vi "Test JKI SM Helper.vi"() -> ()   [LabVIEW 2020]
uses:
  source/JKI State Machine API/source/JKI SM/JKI SM.lvclass/JKI SM.ctl
  source/JKI State Machine API/source/JKI SM/JKI SM.lvclass
  source/JKI State Machine API/tests/TEST JKI State Machine API.lvlib
panel:
  out "error out":errorcluster
  in  "EventStructure?":bool
  # "Run this VI to lauch the JKI State Machine helper on a template VI"
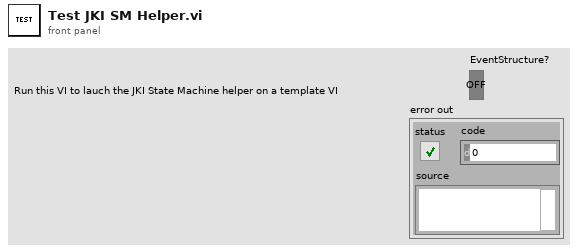
[diagram p1: front panel]
types:
  T1 = cluster{"App.ContextName":string, "VI.Name":string, "Object UID":i32}
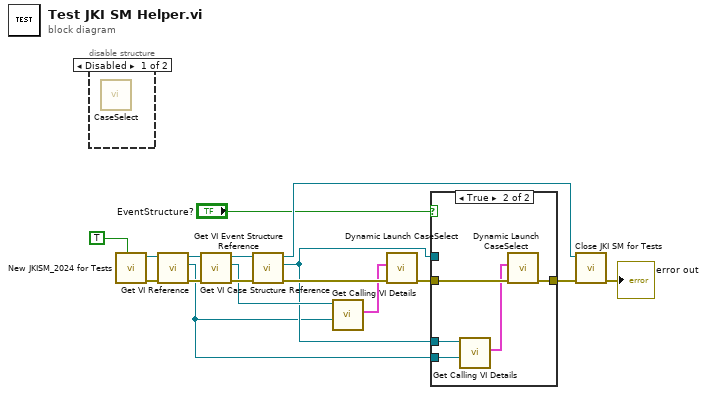
[diagram p0: block diagram]
diagram:
  n1 = disable-structure shown="Disabled" {
    frame Disabled {
      n2 = call "CaseSelect.vi"() -> ()  [unwired: 12 in]
    }
    frame Enabled {
    }
  }
  n3 = call "New JKISM_2024 for Tests.vi"("Open SM FP (for debugging)"=TRUE) -> ("error out"=w16:errorcluster, "JKI SM out"=w17:refnum<class "JKI SM.lvclass">)  [unwired: 9 in]
  n4 = call "Get VI Reference.vi"("error in (no error)"=w16, "JKI SM in"=w17) -> ("error out"=w14:errorcluster, "VI"=w1:refnum<vi>, "JKI SM out"=w15:refnum<class "JKI SM.lvclass">)  [unwired: 7 in]
  n5 = call "Get VI Case Structure Reference.vi"("error in (no error)"=w14, "JKI SM in"=w15) -> ("error out"=w11:errorcluster, "Case Structure ref"=w4:refnum<vi>, "JKI SM out"=w12:refnum<class "JKI SM.lvclass">)  [unwired: 7 in]
  n6 = call "Get VI Event Structure Reference.vi"("error in (no error)"=w11, "JKI SM in"=w12) -> ("error out"=w9:errorcluster, "Event Structure ref"=w2:refnum<vi>, "JKI SM out"=w10:refnum<class "JKI SM.lvclass">)  [unwired: 7 in]
  n7 = call "Get Calling VI Details.vi"("User VI Ref"=w1, "Affected Items"=w4) -> ("Calling VI Details"=w3:T1)  [unwired: 9 in]
  n8 = call "Dynamic Launch CaseSelect.vi"("error in (no error)"=w9, "Owning VI Details"=w3) -> ("error out"=w8:errorcluster)  [unwired: 9 in]
  n9 = case shown="True" "EventStructure?" {
    tunnel: w8 -> [w18 w23]
    tunnel: [w18 w22] -> w7
    tunnel: w2 -> [_ _]
    tunnel: w2 -> [_ w21]
    tunnel: w1 -> [_ w20]
    frame False {
    }
    frame True {
      n10 = call "Get Calling VI Details.vi"("User VI Ref"=w20, "Affected Items"=w21) -> ("Calling VI Details"=w19:T1)  [unwired: 9 in]
      n11 = call "Dynamic Launch CaseSelect.vi"("error in (no error)"=w23, "Owning VI Details"=w19) -> ("error out"=w22:errorcluster)  [unwired: 9 in]
    }
  }
  n12 = call "Close JKI SM for Tests.vi"("error in (no error)"=w7, "JKI SM in"=w10) -> ("error out"=→"error out":errorcluster)  [unwired: 9 in]
